vi "OverlayLabeledRectangleCenterSize.vi"(4 "TextColor":u32(colorbox), 5 "TextSettings":T3={"Desired Font"="Application Font", "Strikeout?"=FALSE, "Italic?"=FALSE, "Underline?"=FALSE, "Outline?"=FALSE, "Shadow?"=FALSE, "Bold?"=FALSE, "Size"=16} {"Size" step=2}, 6 "OverlayColor":u32(colorbox)=16711680, 7 "GroupName":string, 8 "error in":errorcluster, 9 "Text":string, 10 "LabelPosition":T1={"Center-Point"={"X"=0, "Y"=0}, "Size"={"X"=50, "Y"=50}, "Angle"=0.0}, 11 "Image Reference In":T4) -> (0 "error out":errorcluster, 3 "Image Reference Out":T4)   [LabVIEW 2020, in "OpenLvVision_Overlays.lvlib"]
doc: "Overlays an rectangle with text on top of an image."
uses:
  OpenLvVision_Overlays.lvlib
  <vilib>/OpenLvVision/OpenLvVision_Image/Management/TypeDef/OLV Image.ctl
  TypeDefs/TextSettings.ctl
  TypeDefs/LabelPosition.ctl
  TypeDefs/PointI32.ctl
  TypeDefs/RotatedRectangle.ctl
  <vilib>/OpenLvVision/OpenLvVision_Image/Management/OLV Management.lvlib
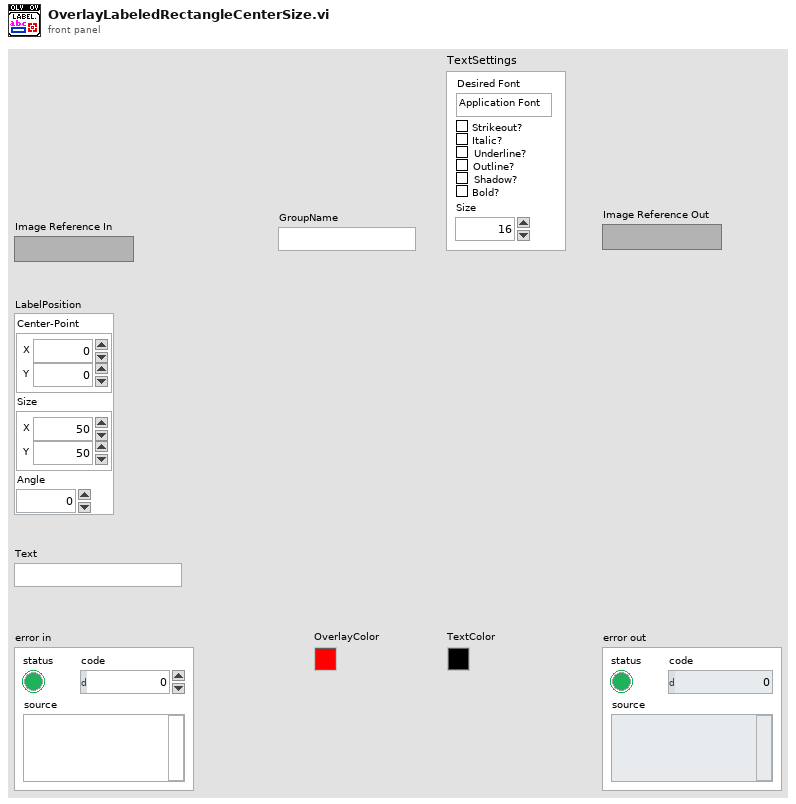
[diagram p1: front panel]
types:
  T1 = typedef "OpenLvVision_Overlays.lvlib/LabelPosition.ctl" = cluster{"Center-Point":T2, "Size":T2, "Angle":dbl}
  T2 = typedef "OpenLvVision_Overlays.lvlib/PointI32.ctl" = cluster{"X":i32, "Y":i32}
  T3 = typedef "OpenLvVision_Overlays.lvlib/TextSettings.ctl" = cluster{"Desired Font":string, "Strikeout?":bool, "Italic?":bool, "Underline?":bool, "Outline?":bool, "Shadow?":bool, "Bold?":bool, "Size":i32}
  T4 = typedef "OLV OpenLvVision_Image.lvlib/OLV Management.lvlib/OLV Image.ctl" = refnum<image>
  T5 = typedef "OpenLvVision_Overlays.lvlib/RotatedRectangle.ctl" = cluster{"TopLeft":T2, "TopRight":T2, "BottomRight":T2, "BottomLeft":T2}
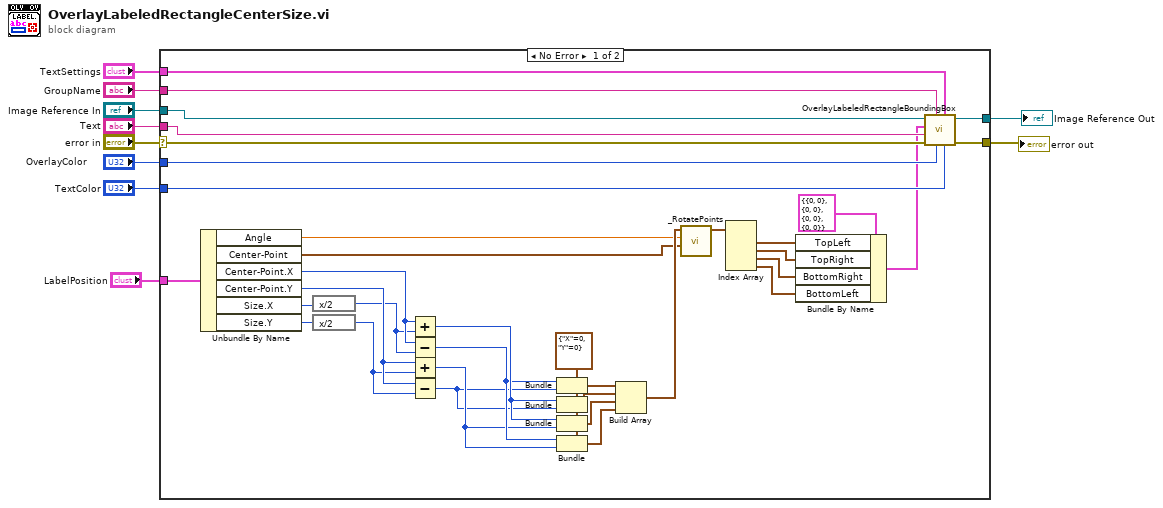
[diagram p0: block diagram]
diagram:
  n1 = case shown="No Error" "error in" {
    selector: "error in" -> [w42 w46]
    tunnel: [w44 w46] -> w9
    tunnel: "Image Reference In" -> [w43 w47]
    tunnel: [w45 w47] -> w8
    tunnel: "GroupName" -> [w41 _]
    tunnel: "OverlayColor" -> [w39 _]
    tunnel: "Text" -> [w37 _]
    tunnel: "TextSettings" -> [w40 _]
    tunnel: "TextColor" -> [w38 _]
    tunnel: "LabelPosition" -> [w15 _]
    frame No Error {
      w29 = T2 {"X"=0, "Y"=0} ("Origin")
      n2 = Unbundle By Name(w15) -> ("Angle"=w11:dbl, "Center-Point"=w12:T2, "Center-Point.X"=w23:i32, "Center-Point.Y"=w22:i32, "Size.X"=w14:i32, "Size.Y"=w13:i32)
      n3 = expression code="x/2"(w14) -> (w20:i32)
      n4 = expression code="x/2"(w13) -> (w21:i32)
      n5 = Add(x=w23, y=w20) -> (x+y=w19:i32)
      n6 = Subtract(x=w23, y=w20) -> (x-y=w18:i32)
      n7 = Add(x=w22, y=w21) -> (x+y=w17:i32)
      n8 = Subtract(x=w22, y=w21) -> (x-y=w16:i32)
      n9 = Bundle(cluster=w29, "X"=w18, "Y"=w16) -> (w28:T2)
      n10 = Bundle(cluster=w29, "X"=w19, "Y"=w16) -> (w27:T2)
      n11 = Bundle(cluster=w29, "X"=w19, "Y"=w17) -> (w26:T2)
      n12 = Bundle(cluster=w29, "X"=w18, "Y"=w17) -> (w25:T2)
      n13 = Build Array(w28, w27, w26, w25) -> (w24:T2[])
      n14 = call "_RotatePoints.vi"("Origin"=w12, "Angle"=w11, "Points in"=w24) -> ("Points out"=w34:T2[])  [unwired: 8 in]
      n15 = Index Array(array=w34) -> (element #1=w33:T2, element #2=w32:T2, element #3=w31:T2, element #4=w30:T2)  [unwired: 4 in]
      n16 = Bundle By Name(cluster=T5 {"TopLeft"={"X"=0, "Y"=0}, "TopRight"={"X"=0, "Y"=0}, "BottomRight"={"X"=0, "Y"=0}, "BottomLeft"={"X"=0, "Y"=0}} ("BoundingBox"), "TopLeft"=w33, "TopRight"=w32, "BottomRight"=w31, "BottomLeft"=w30) -> (w35:T5)
      n17 = call "OverlayLabeledRectangleBoundingBox.vi"("TextColor"=w38, "TextSettings"=w40, "OverlayColor"=w39, "GroupName"=w41, "error in"=w42, "Text"=w37, "BoundingBox"=w35, "Image Reference In"=w43) -> ("error out"=w44:errorcluster, "Image Reference Out"=w45:T4)  [unwired: 2 in]
    }
    frame Error {
    }
  }
  "error out" <- w9
  "Image Reference Out" <- w8
